vi "Host.vi"() -> ()   [LabVIEW 2019]
uses:
  <vilib>/NI VeriStand/Execution/Workspace/NI VeriStand - Get Multiple Channel Values.vi
  <vilib>/NI VeriStand/Execution/Workspace/NI VeriStand - Set Single Channel Value.vi
  <vilib>/NI VeriStand/Execution/Project/NI_VS Project ExecutionAPI.lvlib
  <vilib>/NI VeriStand/Execution/Workspace/NI_VS Workspace ExecutionAPI.lvlib
panel:
  in  "Trigger DMA":bool
  in  "Tab Control":enum32{"Table", "DMA Waveform"}(tab)
  out "Table":string[][](table)
  out "Graph":waveform(dbl)[](graph)
  in  "Exit":bool
  in  "Engine RPM":dbl
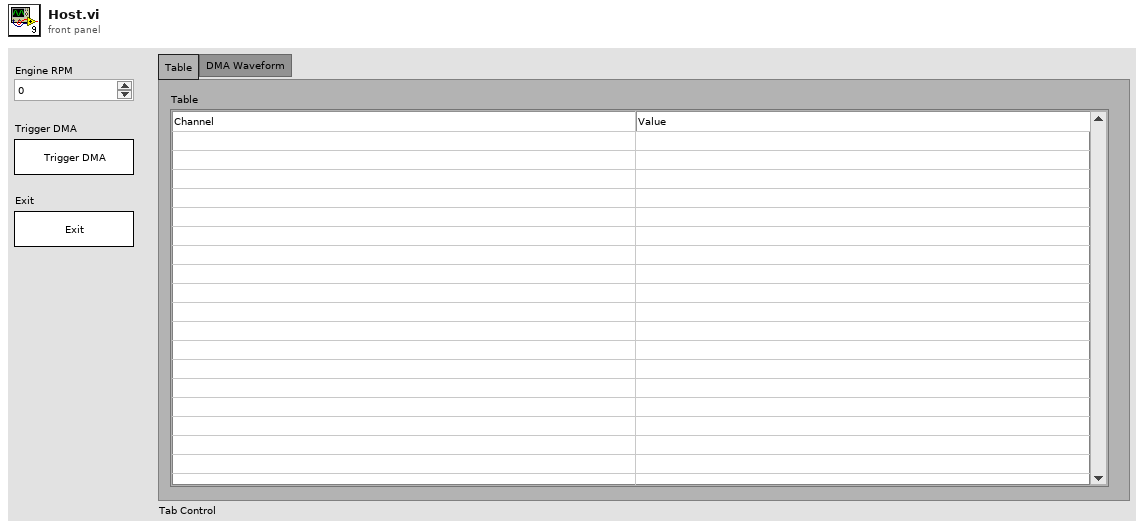
[diagram p1: front panel]
types:
  T1 = typedef "NI_VS Project ExecutionAPI.lvlib/Project Ref.ctl" = refnum<k24>
  T2 = typedef "NI_VS Workspace ExecutionAPI.lvlib/WorkspaceAPI.ctl" = refnum<k24>
  T3 = typedef "NI_VS Workspace ExecutionAPI.lvlib/NodeInfo.ctl" = cluster{"Name":string, "FullPath":string, "Type":string, "IsChannel":bool, "Channel":cluster{"Unit":string, "Readable":bool, "Writable":bool, "Faultable":bool, "Scalable":bool, "RowDim":u32, "ColumnDim":u32, "Value Table Names":string[], "Value Table Values":dbl[]}, "IsWaveform":bool, "Waveform":cluster{"DataType":T4}}
  T4 = typedef "NI_VS Workspace ExecutionAPI.lvlib/Waveform Data Type.ctl" = enum16{"Double", "ComplexDouble"}
  T5 = typedef "NI_VS Waveform Streaming Interface.lvlib/WaveformStreamSpecification.ctl" = refnum<k24>
  T6 = typedef "NI_VS Waveform Streaming Interface.lvlib/Registered Waveform Streams Data Event Refnum (DBL).ctl" = cluster{"Callback Refnum":refnum<k27>, "Data Event":refnum<user-event>, "Event Refnum":refnum<event-registration>, "WaveformDataWatcherDBL":T7}
  T7 = typedef "NI_VS Waveform Streaming Interface.lvlib/WaveformDataWatcherDBL.ctl" = refnum<k24>
  T8 = typedef "NI_VS Waveform Streaming Interface.lvlib/WaveformStreamingAPI.ctl" = refnum<k24>
  T9 = cluster{"Waveform.Refs":T5[], "WaveformStreaming.Event.Refs":T6, "WaveformStreaming.Ref":T8}
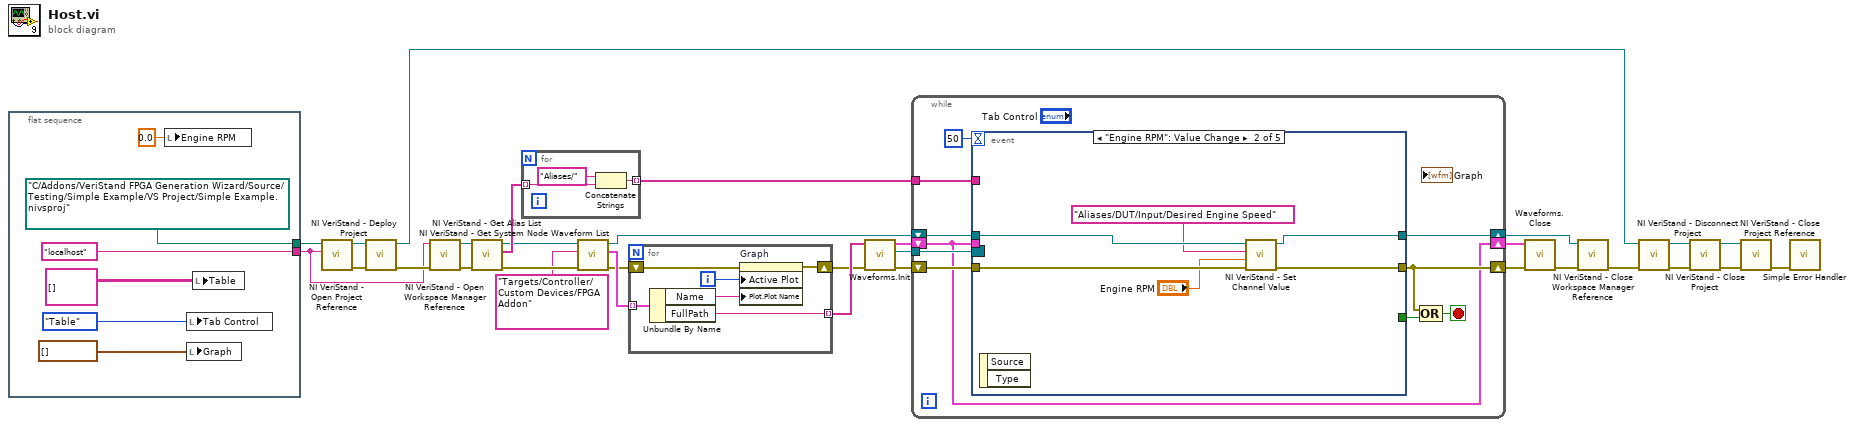
[diagram p0: block diagram]
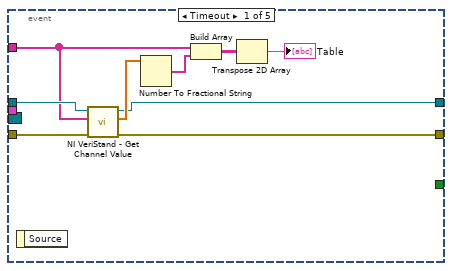
[diagram p2: hidden frame]
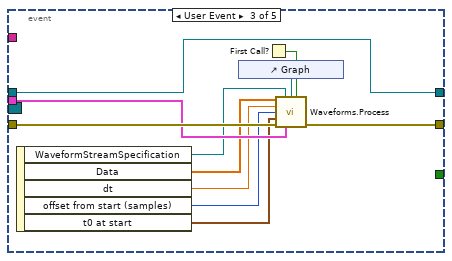
[diagram p3: hidden frame]
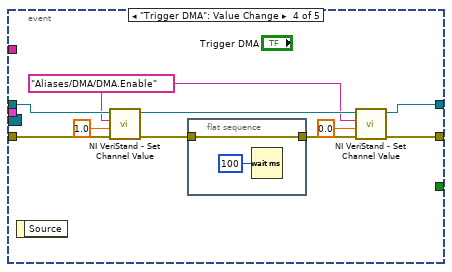
[diagram p4: hidden frame]
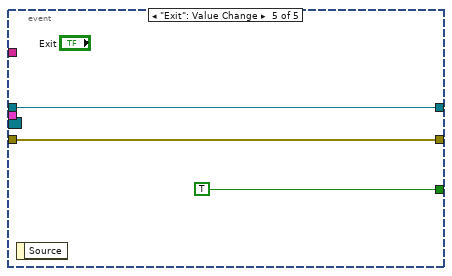
[diagram p5: hidden frame]
diagram:
  n1 = flat-sequence {
    tunnel: [path "C:/Addons/VeriStand FPGA Generation Wizard/Source/Testing/Simple Example/VS Project/Simple Example.nivsproj" ("Project File Path")] -> w29
    tunnel: ["localhost" ("Gateway IP Address (\"\": localhost)")] -> w1
    frame #0 {
      n2 = local write "Engine RPM"(0.0 ("Engine RPM")) -> ()
      n3 = local write "Tab Control"(enum32{"Table", "DMA Waveform"}."Table" ("Tab Control")) -> ()
      n4 = local write "Graph"(waveform(dbl)[] [] ("Graph")) -> ()
      n5 = local write "Table"(string[][] [] ("Table")) -> ()
    }
  }
  n6 = call <vilib>:"NI VeriStand - Open Project Reference.vi"("Gateway IP Address (\"\": localhost)"=w1, "Project File Path"=w29) -> ("error out"=w30:errorcluster, "Project Ref"=w31:T1)  [unwired: 8 in]
  n7 = call <vilib>:"NI VeriStand - Deploy Project.vi"("error in (no error)"=w30, "Project Ref in"=w31) -> ("error out"=w23:errorcluster, "Project Ref out"=w22:T1)  [unwired: 8 in]
  n8 = call <vilib>:"NI VeriStand - Open Workspace Manager Reference.vi"("error in (no error)"=w23, "Gateway IP Address (\"\": localhost)"=w1) -> ("error out"=w27:errorcluster, "WorkspaceManager"=w28:T2)  [unwired: 8 in]
  n9 = call <vilib>:"NI VeriStand - Get Alias List.vi"("error in (no error)"=w27, "WorkspaceManager in"=w28) -> ("error out"=w13:errorcluster, "Aliases"=w21:string[], "WorkspaceManager out"=w11:T2)  [unwired: 6 in, 1 out]
  n10 = for {
    tunnel: w21 -> [w40] mode=indexing
    tunnel: [w38] -> w20 mode=indexing
    n11 = Concatenate Strings("Aliases/" ("string"), w40) -> (w38:string)
  }
  n12 = call <vilib>:"NI VeriStand - Get System Node Waveform List.vi"("error in (no error)"=w13, "StartNode (\"\")"="Targets/Controller/Custom Devices/FPGA Addon" ("StartNode (\"\")"), "WorkspaceManager in"=w11) -> ("error out"=w2:errorcluster, "Waveforms"=w9:T3[], "WorkspaceManager out"=w10:T2)  [unwired: 6 in]
  n13 = for {
    tunnel: w9 -> [w46] mode=indexing
    tunnel: [w45] -> w8 mode=indexing
    shift-right: [w43] -> w3
    shift-left: w2 -> [w41]
    i -> [w42]
    n14 = Unbundle By Name(w46) -> ("Name"=w44:string, "FullPath"=w45:string)
    n15 = property on="Graph" class="WFGraph (strict)"(error in=w41, "Active Plot"=w42, "Plot.Plot Name"=w44) -> (error out=w43:errorcluster)  [unwired: 1 in, 1 out]
  }
  n16 = call "Waveforms.Init.vi"("error in"=w3, "Channel.Paths"=w8) -> ("error out"=w15:errorcluster, "WaveformStreaming.Event"=w14:refnum<event-registration>, "Waveforms"=w7:T9)  [unwired: 7 in]
  n17 = while {
    tunnel: w20 -> [w54]
    shift-right: [w52] -> w25
    shift-left: w10 -> [w55]
    shift-right: [w51] -> w5
    shift-left: w15 -> [w56]
    tunnel: w14 -> [w48]
    shift-right: [w47] -> w6
    shift-left: w7 -> [w47]
    stop <- w49 stop-if-true
    n18 = event shown="[1] \"Engine RPM\": Value Change" {
      selector: w48 -> [_ _ _ _ _]
      dyn-events: _ -> [_ _ _ _ _]
      timeout: 50 -> [_ _ _ _ _]
      tunnel: w56 -> [w65 w71 w82 w92 w97]
      tunnel: w55 -> [w64 w70 w73 w91 w96]
      tunnel: w54 -> [w60 _ _ _ _]
      tunnel: [w58 w68 w73 w87 w96] -> w52
      tunnel: [w57 w69 w75 w88 w97] -> w51
      tunnel: [_ _ _ _ TRUE] -> w50
      tunnel: w47 -> [_ _ w81 _ _]
      event Timeout {
        n19 = event-data() -> ()  [unwired: 1 in, 1 out]
        n20 = call-poly <vilib>:"NI VeriStand - Get Channel Value.vi"("error in (no error)"=w65, "Channels"=w60, "WorkspaceManager in"=w64) -> ("error out"=w57:errorcluster, "Values"=w61:dbl[], "WorkspaceManager out"=w58:T2)  [unwired: 6 in]
        n21 = Number To Fractional String(number=w61) -> (F-format string=w63:string[])  [unwired: 3 in]
        n22 = Build Array(w60, w63) -> (w62:string[][])
        n23 = Transpose 2D Array(2D array=w62) -> (transposed array=→"Table":string[][])
      }
      event "Engine RPM": Value Change {
        n24 = event-data() -> ()  [unwired: 1 in, 2 out]
        n25 = call-poly <vilib>:"NI VeriStand - Set Channel Value.vi"("error in (no error)"=w71, "Value"="Engine RPM", "Channel"="Aliases/DUT/Input/Desired Engine Speed" ("string"), "WorkspaceManager in"=w70) -> ("error out"=w69:errorcluster, "WorkspaceManager out"=w68:T2)  [unwired: 6 in]
      }
      event User Event {
        n26 = event-data() -> ("WaveformStreamSpecification"=w76:T5, "Data"=w80:dbl[], "dt"=w79:dbl, "offset from start (samples)"=w78:u64, "t0 at start"=w77:timestamp)  [unwired: 1 in]
        n27 = control-ref of="Graph"() -> (w74:refnum<vi>)
        n28 = First Call?() -> (First Call?: T/F=w72:bool)
        n29 = call "Waveforms.Process.vi"("Data"=w80, "Waveform.Ref"=w76, "WaveformGraph.Ref"=w74, "Reset?"=w72, "dt"=w79, "offset from start (samples)"=w78, "t0 at start"=w77, "error in (no error)"=w82, "Waveforms"=w81) -> ("error out"=w75:errorcluster)  [unwired: 6 in]
      }
      event "Trigger DMA": Value Change {
        w84 = "Aliases/DMA/DMA.Enable" ("string")
        n30 = event-data() -> ()  [unwired: 1 in, 1 out]
        n31 = call-poly <vilib>:"NI VeriStand - Set Channel Value.vi"("error in (no error)"=w92, "Value"=1.0, "Channel"=w84, "WorkspaceManager in"=w91) -> ("error out"=w85:errorcluster, "WorkspaceManager out"=w89:T2)  [unwired: 6 in]
        n32 = flat-sequence {
          tunnel: [w93] -> w86
          tunnel: w85 -> [w93]
          frame #0 {
            n33 = Wait (ms)(milliseconds to wait=u32 100) -> ()  [unwired: 1 out]
          }
        }
        n34 = call-poly <vilib>:"NI VeriStand - Set Channel Value.vi"("error in (no error)"=w86, "Value"=0.0, "Channel"=w84, "WorkspaceManager in"=w89) -> ("error out"=w88:errorcluster, "WorkspaceManager out"=w87:T2)  [unwired: 6 in]
      }
      event "Exit": Value Change {
        n35 = event-data() -> ()  [unwired: 1 in, 1 out]
      }
    }
    n36 = Compound Arithmetic op=OR(w51, w50) -> (w49:bool)
  }
  n37 = call "Waveforms.Close.vi"("error in (no error)"=w5, "Waveforms"=w6) -> ("error out"=w4:errorcluster)  [unwired: 9 in]
  n38 = call <vilib>:"NI VeriStand - Close Workspace Manager Reference.vi"("error in (no error)"=w4, "WorkspaceManager"=w25) -> ("error out"=w24:errorcluster)  [unwired: 9 in]
  n39 = call <vilib>:"NI VeriStand - Disconnect Project.vi"("error in (no error)"=w24, "Project Ref in"=w22) -> ("error out"=w18:errorcluster, "Project Ref out"=w26:T1)  [unwired: 8 in]
  n40 = call <vilib>:"NI VeriStand - Close Project.vi"("error in (no error)"=w18, "Project Ref in"=w26) -> ("error out"=w17:errorcluster, "Project Ref out"=w19:T1)  [unwired: 8 in]
  n41 = call <vilib>:"NI VeriStand - Close Project Reference.vi"("error in (no error)"=w17, "Project Ref"=w19) -> ("error out"=w16:errorcluster)  [unwired: 9 in]
  n42 = call <vilib>:"Simple Error Handler.vi"("error in (no error)"=w16) -> ()  [unwired: 4 in, 5 out]
